vi "SMTP Email Close Session.vi"(4 "error in (no error)":errorcluster caption="entrée d'erreur (pas d'erreur)", 7 "smtp session":T1 caption="session smtp") -> (0 "error out":errorcluster caption="sortie d'erreur", 3 "smtp session out":T1 caption="session smtp en sortie")   [LabVIEW 2022 SP3, in "Copie de NI_SMTPEmail.lvlib"]
doc: "Ce VI envoie la commande QUIT au serveur SMTP puis ferme la connexion TCP spécifiée avec \"ID de connexion\". Il propage toute erreur rencontrée pendant ou avant l'appel de ce VI à travers le cluster 'sortie d'erreur'."
uses:
  Copie de NI_SMTPEmail.lvlib
  SMTP Email Session.ctl
panel:
  in  "tcp connection":refnum<k5> caption="connexion tcp"
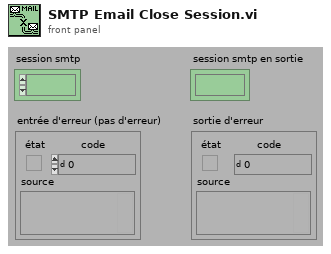
[diagram p1: front panel]
types:
  T1 = typedef "Copie de NI_SMTPEmail.lvlib/SMTP Email Session.ctl" = refnum<k1>
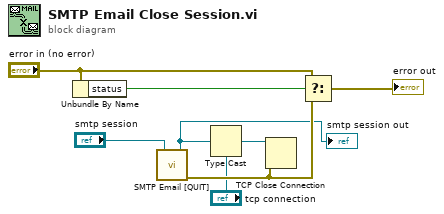
[diagram p0: block diagram]
diagram:
  n1 = Unbundle By Name("error in (no error)") -> ("status"=w8:bool)
  n2 = call "SMTP Email [QUIT].vi"("smtp session"="smtp session") -> ("error out"=w5:errorcluster, "smtp session out"=w4:T1)  [unwired: 3 in, 2 out]
  "smtp session out" <- w4
  n3 = Type Cast(type="tcp connection", x=w4) -> (*(type *) &x=w3:refnum<k5>)
  n4 = TCP Close Connection(connection ID=w3, error in (no error)=w5) -> ()  [unwired: 1 in, 2 out]
  n5 = Select(t="error in (no error)", s=w8, f=w5) -> (s? t:f=→"error out":errorcluster)
